vi "VIH Utility - VISRV - Get Nested Control Refnums.vi"(5 "array element (T)":bool=TRUE, 7 "cluster members (T)":bool=TRUE, 8 "error in":errorcluster, 10 "include original Ctl Refnum (F)":bool, 11 "Ctl Refnum":refnum<vi>) -> (0 "error out":errorcluster, 2 "nested Ctl Refnums":refnum<vi>[](array[refnum]), 3 "dup Ctl Refnum":refnum<vi>)   [LabVIEW 2014]
doc: "::: VI Helpeks :::\nCopyright (c) 2000-2026 Konstantin Shifershteyn. All rights reserved."
panel:
  # "VI Helpeks\nCopyright (c) 2012-2026 Konstantin Shifershteyn"
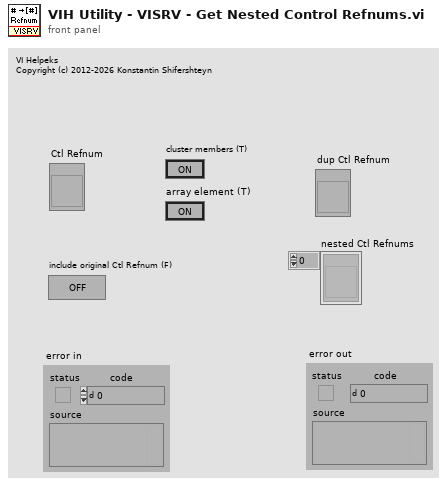
[diagram p1: front panel]
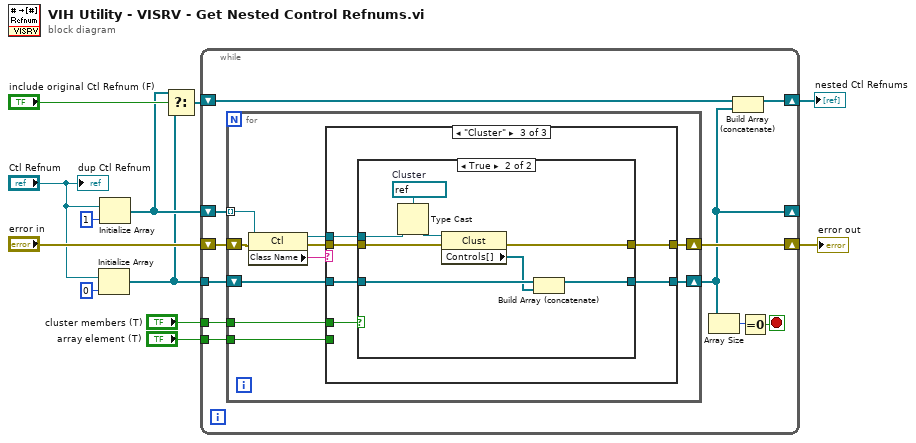
[diagram p0: block diagram]
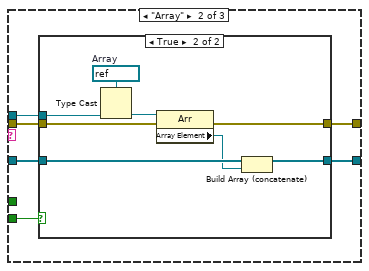
[diagram p3: hidden frame]
diagram:
  n1 = Initialize Array("Ctl Refnum", 0 ("dimension size")) -> (w4:refnum<vi>[])
  n2 = Initialize Array("Ctl Refnum", 1 ("dimension size")) -> (w5:refnum<vi>[])
  n3 = Select(t=w5, s="include original Ctl Refnum (F)", f=w4) -> (s? t:f=w3:refnum<vi>[])
  n4 = while {
    shift-right: [w17] -> _
    shift-left: w5 -> [w16]
    shift-right: [w22] -> w12
    shift-left: w3 -> [w23]
    shift-right: [w18] -> w11
    shift-left: "error in" -> [w19]
    tunnel: w4 -> [w15]
    tunnel: "cluster members (T)" -> [w14]
    tunnel: "array element (T)" -> [w13]
    stop <- w20 stop-if-true
    n5 = for {
      tunnel: w16 -> [w33] mode=indexing
      shift-right: [w28] -> w17
      shift-left: w15 -> [w29]
      shift-right: [w26] -> w18
      shift-left: w19 -> [w27]
      tunnel: w14 -> [w25]
      tunnel: w13 -> [w24]
      n6 = property class="Ctl"(reference=w33, error in=w27) -> (reference out=w31:refnum<vi>, error out=w30:errorcluster, "Class Name"=w32:string)
      n7 = case shown="\"Cluster\"" w32 {
        tunnel: w31 -> [_ w41 w54]
        tunnel: w30 -> [w34 w40 w53]
        tunnel: w29 -> [w35 w39 w57]
        tunnel: [w35 w38 w56] -> w28
        tunnel: [w34 w37 w55] -> w26
        tunnel: w25 -> [_ _ w52]
        tunnel: w24 -> [_ w36 _]
        frame Default {
        }
        frame "Array" {
          n8 = case shown="True" w36 {
            tunnel: w41 -> [_ w46]
            tunnel: w40 -> [w42 w47]
            tunnel: w39 -> [w43 w51]
            tunnel: [w43 w50] -> w38
            tunnel: [w42 w49] -> w37
            frame False {
            }
            frame True {
              w44 = refnum<vi> refnum  # Array
              n9 = Type Cast(type=w44, x=w46) -> (*(type *) &x=w45:refnum<vi>)
              n10 = property class="Arr"(reference=w45, error in=w47) -> (error out=w49:errorcluster, "Array Element"=w48:refnum<vi>)  [unwired: 1 out]
              n11 = Build Array (concatenate)(w51, w48) -> (w50:refnum<vi>[])
            }
          }
        }
        frame "Cluster" {
          n12 = case shown="True" w52 {
            tunnel: w57 -> [w59 w67]
            tunnel: [w59 w66] -> w56
            tunnel: [w58 w65] -> w55
            tunnel: w54 -> [_ w63]
            tunnel: w53 -> [w58 w60]
            frame False {
            }
            frame True {
              w62 = refnum<vi> refnum  # Cluster
              n13 = Type Cast(type=w62, x=w63) -> (*(type *) &x=w61:refnum<vi>)
              n14 = property class="Clust"(reference=w61, error in=w60) -> (error out=w65:errorcluster, "Controls[]"=w64:refnum<vi>[])  [unwired: 1 out]
              n15 = Build Array (concatenate)(w67, w64) -> (w66:refnum<vi>[])
            }
          }
        }
      }
    }
    n16 = Array Size(array=w17) -> (size(s)=w21:i32)
    n17 = Build Array (concatenate)(w23, w17) -> (w22:refnum<vi>[])
    n18 = Equal To 0?(x=w21) -> (x = 0?=w20:bool)
  }
  "nested Ctl Refnums" <- w12
  "error out" <- w11
  "dup Ctl Refnum" <- "Ctl Refnum"
